vi "Enemy_Walk.vi"(0 "Tiles":u8[][](array[numeric]), 5 "Enemy":T1={"Kind"=0, "X10"=0, "Y10"=0, "Dir"=1, "Mode"=0}, 7 "Speed":i32, 9 "Random":i32, 11 "error in":errorcluster) -> (4 "X10":i32, 6 "Dir":i32, 8 "Mode":i32, 15 "error out":errorcluster)   [LabVIEW 2020, in "GH_Engine.lvlib"]
doc: "One step of a walking enemy: turns at walls, doors, edges, ladder holes (skull), vanishing floors and the room edge; a spider walks over ladder tops and, crossing a tile border at a ladder or rope, may start to climb up or down (Random). Inline subVI of Enemies_Step."
uses:
  GH_Engine.lvlib
  Level/GH_Level.lvlib
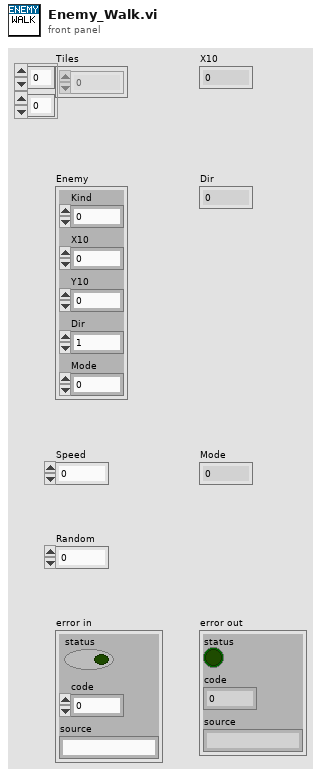
[diagram p1: front panel]
types:
  T1 = cluster{"Kind":i32, "X10":i32, "Y10":i32, "Dir":i32, "Mode":i32}
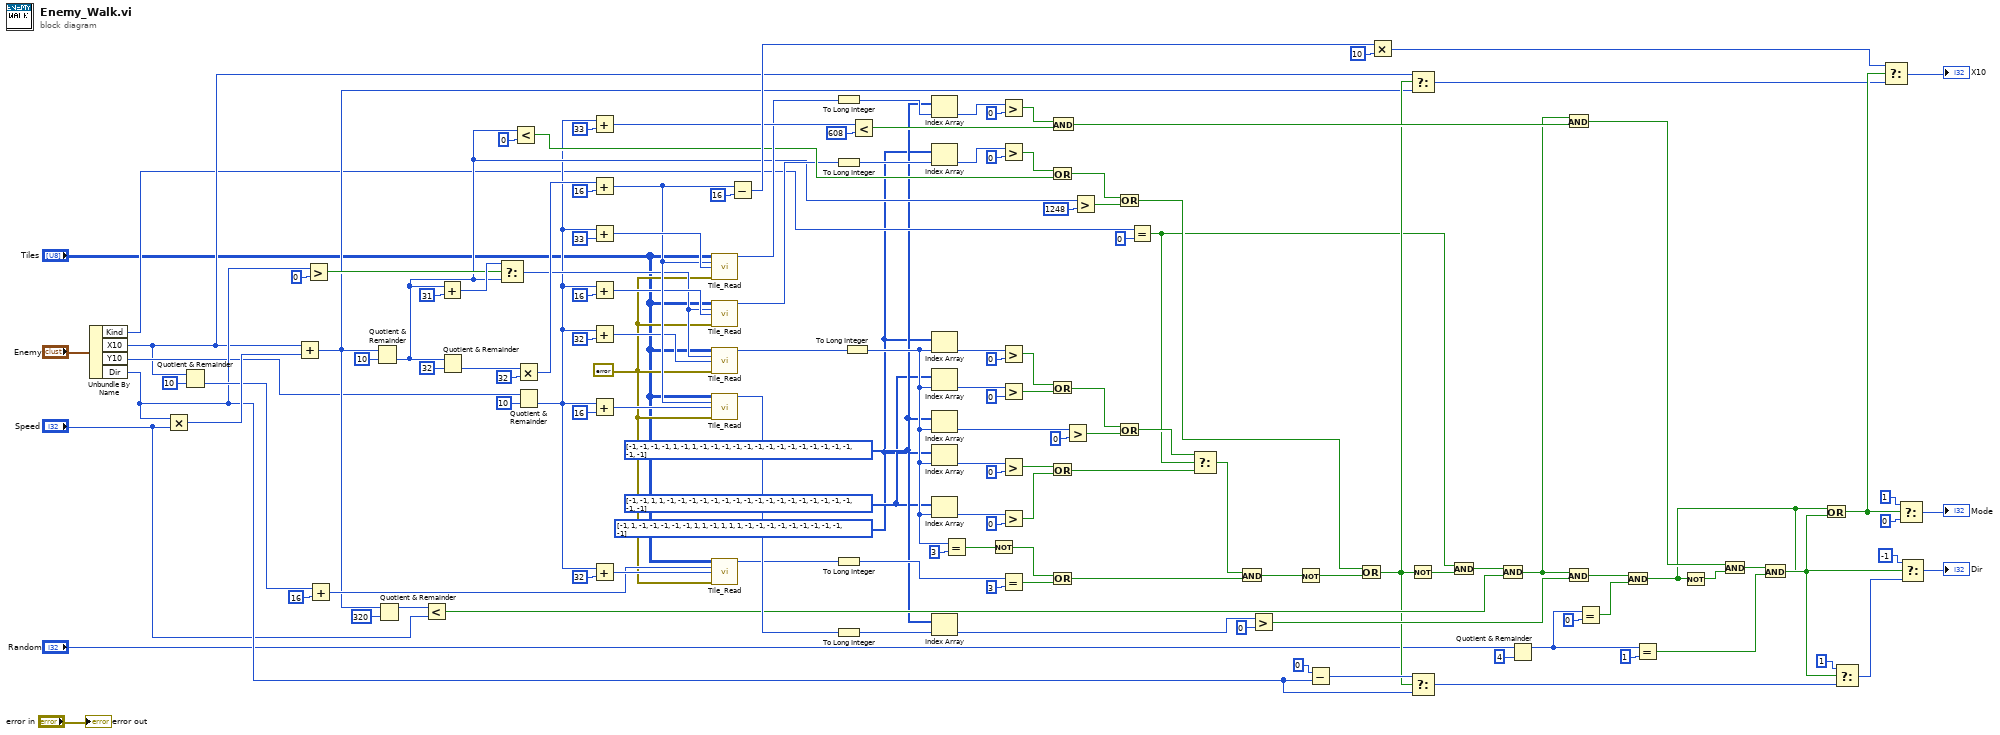
[diagram p0: block diagram]
diagram:
  w13 = errorcluster {"status"=FALSE, "code"=0, "source"=""} ("no error")
  w8 = i32[] [-1, -1, -1, -1, 1, -1, 1, -1, -1, -1, -1, -1, -1, -1, -1, -1, -1, -1, -1, -1, -1, -1, -1] ("Ladder or rope")
  w7 = i32[] [-1, -1, 1, 1, -1, -1, -1, -1, -1, -1, -1, -1, -1, -1, -1, -1, -1, -1, -1, -1, -1, -1, -1] ("Thin floor")
  w6 = i32[] [-1, 1, -1, -1, -1, -1, -1, 1, 1, -1, 1, 1, 1, -1, -1, -1, -1, -1, -1, -1, -1, -1, -1] ("Solid")
  n1 = Unbundle By Name("Enemy") -> ("Kind"=w9:i32, "X10"=w10:i32, "Y10"=w11:i32, "Dir"=w12:i32)
  n2 = Multiply(x=w12, y="Speed") -> (x*y=w20:i32)
  n3 = Quotient & Remainder(x=w10, y=10) -> (floor(x/y)=w15:i32)  [unwired: 1 out]
  n4 = Add(x=w10, y=w20) -> (x+y=w21:i32)
  n5 = Greater?(x=w12, y=0) -> (0:w25:bool)
  n6 = Add(x=w15, y=16) -> (x+y=w36:i32)
  n7 = Quotient & Remainder(x=w21, y=10) -> (floor(x/y)=w23:i32)  [unwired: 1 out]
  n8 = Quotient & Remainder(x=w21, y=320) -> (x-y*floor(x/y)=w86:i32)  [unwired: 1 out]
  n9 = Less?(x=w86, y="Speed") -> (x < y?=w87:bool)
  n10 = Add(x=w23, y=31) -> (x+y=w27:i32)
  n11 = Quotient & Remainder(x=w23, y=32) -> (floor(x/y)=w91:i32)  [unwired: 1 out]
  n12 = Select(t=w27, s=w25, f=w23) -> (s? t:f=w28:i32)
  n13 = Less?(x=w23, y=0) -> (x < y?=w73:bool)
  n14 = Multiply(x=w91, y=32) -> (x*y=w93:i32)
  n15 = Quotient & Remainder(x=w11, y=10) -> (floor(x/y)=w17:i32)  [unwired: 1 out]
  n16 = Add(x=w17, y=33) -> (x+y=w111:i32)
  n17 = Add(x=w93, y=16) -> (x+y=w95:i32)
  n18 = Add(x=w17, y=33) -> (x+y=w104:i32)
  n19 = Add(x=w17, y=16) -> (x+y=w66:i32)
  n20 = Add(x=w17, y=32) -> (x+y=w30:i32)
  n21 = Add(x=w17, y=16) -> (x+y=w97:i32)
  n22 = Add(x=w17, y=32) -> (x+y=w38:i32)
  n23 = call "Tile_Read.vi"("Tiles"="Tiles", "X"=w95, "Y"=w104, "error in"=w13) -> ("Tile"=w105:u8)  [unwired: 10 in, 1 out]
  n24 = call "Tile_Read.vi"("Tiles"="Tiles", "X"=w28, "Y"=w66, "error in"=w13) -> ("Tile"=w67:u8)  [unwired: 10 in, 1 out]
  n25 = call "Tile_Read.vi"("Tiles"="Tiles", "X"=w28, "Y"=w30, "error in"=w13) -> ("Tile"=w31:u8)  [unwired: 10 in, 1 out]
  n26 = call "Tile_Read.vi"("Tiles"="Tiles", "X"=w95, "Y"=w97, "error in"=w13) -> ("Tile"=w98:u8)  [unwired: 10 in, 1 out]
  n27 = call "Tile_Read.vi"("Tiles"="Tiles", "X"=w36, "Y"=w38, "error in"=w13) -> ("Tile"=w39:u8)  [unwired: 10 in, 1 out]
  n28 = Subtract(x=w95, y=16) -> (x-y=w129:i32)
  n29 = To Long Integer(number=w105) -> (32bit integer=w106:i32)
  n30 = To Long Integer(number=w67) -> (32bit integer=w68:i32)
  n31 = To Long Integer(number=w39) -> (32bit integer=w40:i32)
  n32 = To Long Integer(number=w98) -> (32bit integer=w99:i32)
  n33 = To Long Integer(number=w31) -> (32bit integer=w32:i32)
  n34 = Less?(x=w111, y=608) -> (x < y?=w113:bool)
  n35 = Index Array(array=w8, index=w106) -> (element=w107:i32)
  n36 = Index Array(array=w6, index=w68) -> (element=w69:i32)
  n37 = Index Array(array=w6, index=w32) -> (element=w43:i32)
  n38 = Index Array(array=w7, index=w32) -> (element=w46:i32)
  n39 = Index Array(array=w8, index=w32) -> (element=w49:i32)
  n40 = Index Array(array=w6, index=w32) -> (element=w54:i32)
  n41 = Index Array(array=w7, index=w32) -> (element=w57:i32)
  n42 = Index Array(array=w8, index=w99) -> (element=w100:i32)
  n43 = Equal?(x=w32, y=3) -> (x = y?=w34:bool)
  n44 = Not(x=w34) -> (.not. x?=w62:bool)
  n45 = Greater?(x=w107, y=0) -> (0:w109:bool)
  n46 = Greater?(x=w69, y=0) -> (0:w71:bool)
  n47 = Greater?(x=w43, y=0) -> (0:w45:bool)
  n48 = Greater?(x=w46, y=0) -> (0:w48:bool)
  n49 = Greater?(x=w54, y=0) -> (0:w56:bool)
  n50 = Greater?(x=w57, y=0) -> (0:w59:bool)
  n51 = Equal?(x=w40, y=3) -> (x = y?=w42:bool)
  n52 = Or(x=w71, y=w73) -> (x .or. y?=w77:bool)
  n53 = Or(x=w45, y=w48) -> (x .or. y?=w52:bool)
  n54 = Or(x=w56, y=w59) -> (x .or. y?=w60:bool)
  n55 = Or(x=w62, y=w42) -> (x .or. y?=w63:bool)
  n56 = And(x=w109, y=w113) -> (x .and. y?=w114:bool)
  n57 = Greater?(x=w49, y=0) -> (0:w51:bool)
  n58 = Greater?(x=w23, y=1248) -> (0:w75:bool)
  n59 = Or(x=w77, y=w75) -> (x .or. y?=w78:bool)
  n60 = Or(x=w52, y=w51) -> (x .or. y?=w53:bool)
  n61 = Equal?(x=w9, y=0) -> (x = y?=w19:bool)
  n62 = Select(t=w53, s=w19, f=w60) -> (s? t:f=w61:bool)
  n63 = And(x=w61, y=w63) -> (x .and. y?=w64:bool)
  n64 = Greater?(x=w100, y=0) -> (0:w102:bool)
  n65 = Not(x=w64) -> (.not. x?=w76:bool)
  n66 = Subtract(x=0, y=w12) -> (x-y=w82:i32)
  n67 = Or(x=w78, y=w76) -> (x .or. y?=w79:bool)
  n68 = Multiply(x=w129, y=10) -> (x*y=w131:i32)
  n69 = Not(x=w79) -> (.not. x?=w84:bool)
  n70 = Select(t=w10, s=w79, f=w21) -> (s? t:f=w80:i32)
  n71 = Select(t=w82, s=w79, f=w12) -> (s? t:f=w83:i32)
  n72 = And(x=w19, y=w84) -> (x .and. y?=w88:bool)
  n73 = And(x=w88, y=w87) -> (x .and. y?=w89:bool)
  n74 = Quotient & Remainder(x="Random", y=4) -> (x-y*floor(x/y)=w116:i32)  [unwired: 1 out]
  n75 = And(x=w89, y=w114) -> (x .and. y?=w124:bool)
  n76 = And(x=w89, y=w102) -> (x .and. y?=w119:bool)
  n77 = Equal?(x=w116, y=0) -> (x = y?=w118:bool)
  n78 = And(x=w119, y=w118) -> (x .and. y?=w120:bool)
  n79 = Equal?(x=w116, y=1) -> (x = y?=w123:bool)
  n80 = Not(x=w120) -> (.not. x?=w121:bool)
  n81 = And(x=w124, y=w121) -> (x .and. y?=w125:bool)
  n82 = And(x=w125, y=w123) -> (x .and. y?=w126:bool)
  n83 = Or(x=w120, y=w126) -> (x .or. y?=w127:bool)
  n84 = Select(t=1, s=w126, f=w83) -> (s? t:f=w135:i32)
  n85 = Select(t=w131, s=w127, f=w80) -> (s? t:f=→"X10":i32)
  n86 = Select(t=1, s=w127, f=0) -> (s? t:f=→"Mode":i32)
  n87 = Select(t=-1, s=w120, f=w135) -> (s? t:f=→"Dir":i32)
  "error out" <- "error in"
